vi "Test_Driver.vi"() -> ()   [LabVIEW 2026]
doc: "Use this template to build a VI to use as a subVI."
panel:
  out "error out":errorcluster
  out "Words":u16[](array[numeric])
  in  "Read Count":u16
  in  "Read D":u16
  in  "Write Value":u16
  in  "Write D":u16
  in  "Resource (text)":string
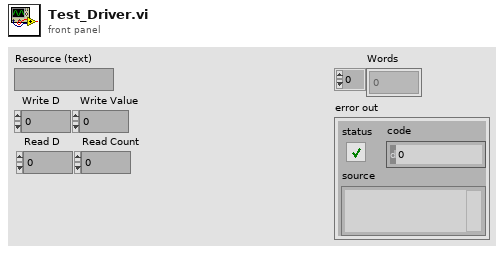
[diagram p1: front panel]
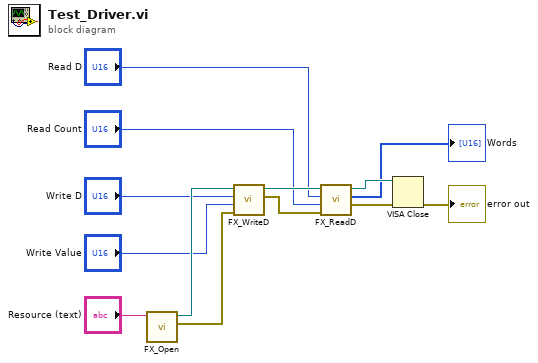
[diagram p0: block diagram]
diagram:
  n1 = call "FX_Open.vi"("Resource"="Resource (text)") -> ("error out"=w11:errorcluster, "VISA out"=w12:refnum<visa-resource-name>)  [unwired: 9 in]
  n2 = call "FX_WriteD.vi"("error in (no error)"=w11, "Value"="Write Value", "D"="Write D", "VISA in"=w12) -> ("error out"=w9:errorcluster, "VISA out"=w10:refnum<visa-resource-name>)  [unwired: 6 in]
  n3 = call "FX_ReadD.vi"("error in (no error)"=w9, "Count"="Read Count", "D"="Read D", "VISA in"=w10) -> ("error out"=w7:errorcluster, "Words"=→"Words":u16[], "VISA out"=w8:refnum<visa-resource-name>)  [unwired: 5 in]
  n4 = VISA Close(VISA resource name=w8, error in (no error)=w7) -> (error out=→"error out":errorcluster)
